vi "menu options.vi"(8 "error in":errorcluster, 9 "VI ref":refnum<vi>, 11 "menu ref in":refnum<k9>) -> (0 "error out":errorcluster, 3 "menu ref out":refnum<k9>)   [LabVIEW 2013, in "Standard Editor.lvlib"]
uses:
  Standard Editor.lvlib
  <vilib>/Utility/miscctls.llb/LVMenuShortCut.ctl
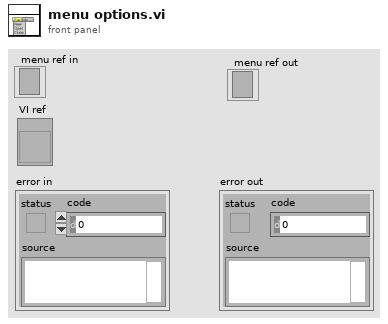
[diagram p1: front panel]
types:
  T1 = typedef "LVMenuShortCut.ctl" = cluster{"Include Shift Key?":bool, "Include Ctrl Key?":bool, "Shortcut Key":string}
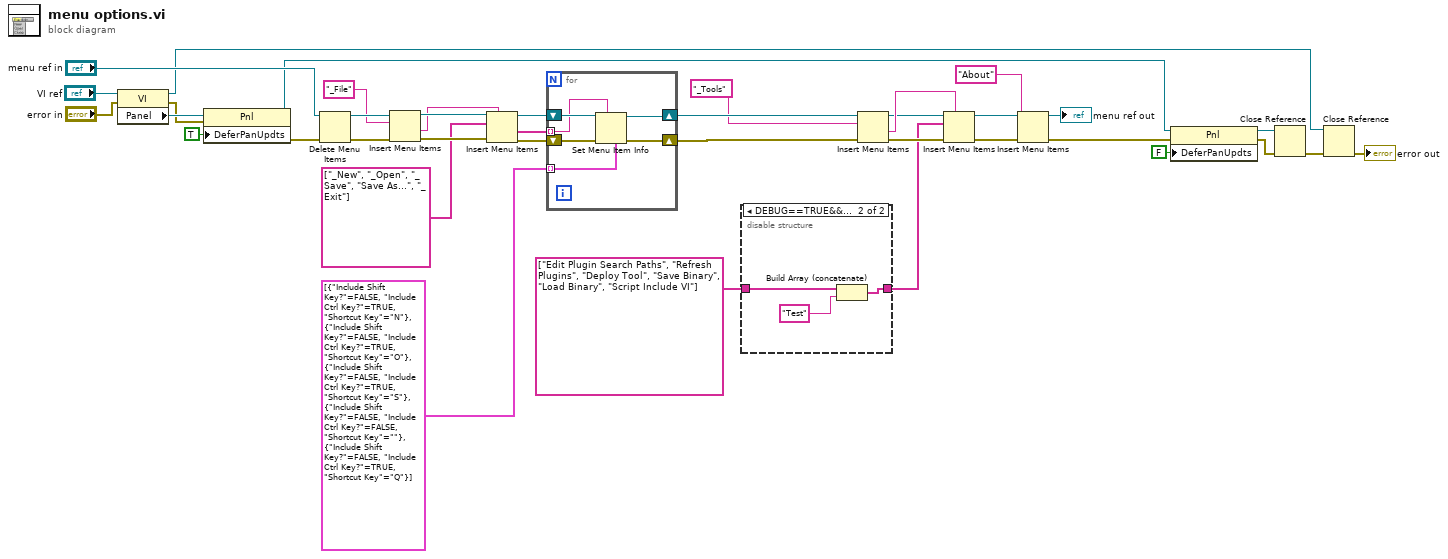
[diagram p0: block diagram]
diagram:
  n1 = property class="VI"(reference="VI ref", error in="error in") -> (reference out=w19:refnum<vi>, error out=w15:errorcluster, "Panel"=w18:refnum<vi>)
  n2 = property class="Pnl"(reference=w18, error in=w15, "DeferPanUpdts"=TRUE ("Defer Panel Updates")) -> (reference out=w12:refnum<vi>, error out=w14:errorcluster)
  n3 = Delete Menu Items(6:w14, 9:"menu ref in") -> (0:w33:errorcluster, 3:w37:refnum<k9>)  [unwired: 2 in]
  n4 = Insert Menu Items(6:w33, 8:"_File", 9:w37) -> (0:w32:errorcluster, 1:w34:string, 3:w35:refnum<k9>)  [unwired: 3 in]
  n5 = Insert Menu Items(5:w34, 6:w32, 8:string[] ["_New", "_Open", "_Save", "Save As...", "_Exit"] ("item names"), 9:w35) -> (0:w29:errorcluster, 1:w28:string[], 3:w30:refnum<k9>)  [unwired: 2 in]
  n6 = for {
    shift-right: [w42] -> w26
    shift-left: w30 -> [w44]
    tunnel: w28 -> [w41] mode=indexing
    tunnel: T1[] [{"Include Shift Key?"=FALSE, "Include Ctrl Key?"=TRUE, "Shortcut Key"="N"}, {"Include Shift Key?"=FALSE, "Include Ctrl Key?"=TRUE, "Shortcut Key"="O"}, {"Include Shift Key?"=FALSE, "Include Ctrl Key?"=TRUE, "Shortcut Key"="S"}, {"Include Shift Key?"=FALSE, "Include Ctrl Key?"=FALSE, "Shortcut Key"=""}, {"Include Shift Key?"=FALSE, "Include Ctrl Key?"=TRUE, "Shortcut Key"="Q"}] -> [w39] mode=indexing
    shift-right: [w40] -> w25
    shift-left: w29 -> [w43]
    n7 = Set Menu Item Info(4:w39, 7:w41, 8:w43, 11:w44) -> (0:w40:errorcluster, 3:w42:refnum<k9>)  [unwired: 3 in]
  }
  n8 = disable-structure shown="DEBUG==TRUE&&RUN_TIME_ENGINE==False" {
    disable-tunnel: [w45 w47] -> w7
    disable-tunnel: string[] ["Edit Plugin Search Paths", "Refresh Plugins", "Deploy Tool", "Save Binary", "Load Binary", "Script Include VI"] ("item names") -> [w45 w48]
    frame condition #0 {
    }
    frame condition #1 (active) {
      n9 = Build Array (concatenate)(w48, "Test") -> (w47:string[])
    }
  }
  n10 = Insert Menu Items(6:w25, 8:"_Tools", 9:w26) -> (0:w23:errorcluster, 1:w24:string, 3:w22:refnum<k9>)  [unwired: 3 in]
  n11 = Insert Menu Items(5:w24, 6:w23, 8:w7, 9:w22) -> (0:w3:errorcluster, 3:w5:refnum<k9>)  [unwired: 2 in, 1 out]
  n12 = Insert Menu Items(6:w3, 8:"About", 9:w5) -> (0:w2:errorcluster, 3:→"menu ref out":refnum<k9>)  [unwired: 3 in, 1 out]
  n13 = property class="Pnl"(reference=w12, error in=w2, "DeferPanUpdts"=FALSE ("Defer Panel Updates")) -> (reference out=w11:refnum<vi>, error out=w10:errorcluster)
  n14 = Close Reference(reference=w11, error in (no error)=w10) -> (error out=w9:errorcluster)
  n15 = Close Reference(reference=w19, error in (no error)=w9) -> (error out=→"error out":errorcluster)
